vi "Add Subscriber.vi"(8 "error in (no error)":errorcluster, 10 "New FIFO Instance Config":T2 {"Custom Data" format="%.0x"}, 11 "CIF_CIPC_Chn in":refnum<class "CIF_Iceoryx_Chn.lvclass">) -> (0 "error out":errorcluster, 2 "New FIFO Instance":T1 {"Custom Data" format="%.0x"}, 3 "CIF_CIPC_Chn out":refnum<class "CIF_Iceoryx_Chn.lvclass">)   [LabVIEW 2021, in "CIF_Iceoryx_Chn.lvclass"]
uses:
  CIF_Iceoryx_Chn.lvclass
  CIF_Iceoryx_Chn.lvclass/CIF_Iceoryx_Chn.ctl
  ChannelCommon/typedef/New FIFO Instance Response.ctl
  ChannelCommon/ChannelCommon.lvlib
  CIFChannels/CIFChannels.lvclass
  D:/dev/Packages/CIF_Channels_Core/src/CIFChannels/CIFChannels.lvclass
  D:/dev/Packages/CIF_Channels_Core/src/Iceorxy_Channels/CIF_Iceoryx_Chan/CIF_Iceoryx_Chn.lvclass
  ChannelCommon/typedef/New FIFO Instance Configuration.ctl
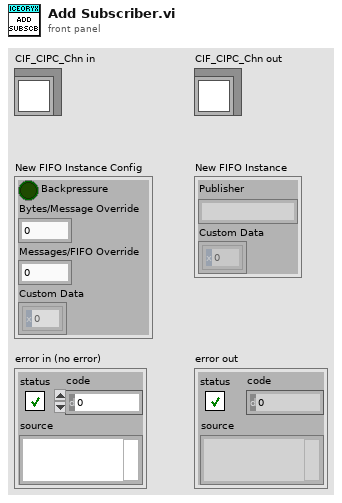
[diagram p1: front panel]
types:
  T1 = typedef "ChannelCommon.lvlib/New FIFO Instance Response.ctl" = cluster{"Publisher":string, "Custom Data":u8[]}
  T2 = typedef "ChannelCommon.lvlib/New FIFO Instance Configuration.ctl" = cluster{"Backpressure":bool, "Bytes/Message Override":u32, "Messages/FIFO Override":u32, "Custom Data":u8[]}
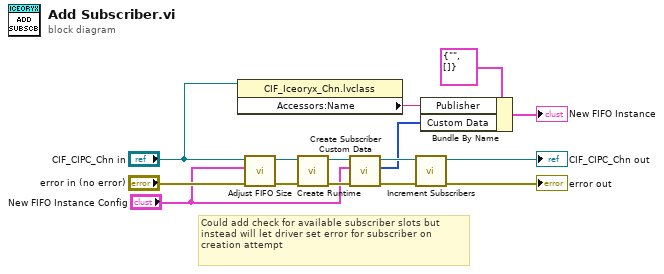
[diagram p0: block diagram]
diagram:
  # "Could add check for available subscriber slots but instead will let driver set error for subscriber on creation attempt"
  n1 = property class="CIF_Iceoryx_Chn.lvclass"(reference="CIF_CIPC_Chn in") -> ("Accessors:Name"=w7:string)  [unwired: 1 in, 2 out]
  n2 = call-dynamic "Adjust FIFO Size.vi"("error in (no error)"="error in (no error)", "New FIFO Instance Config"="New FIFO Instance Config", "CIF_CIPC_Chn in"="CIF_CIPC_Chn in") -> ("error out"=w8:errorcluster, "CIF_CIPC_Chn out"=w9:refnum<class "CIF_Iceoryx_Chn.lvclass">)  [unwired: 7 in]
  n3 = call-dynamic "Create Runtime.vi"("error in (no error)"=w8, "CIFChannels in"=w9) -> ("error out"=w5:errorcluster, "CIFChannels out"=w6:refnum<class "CIF_Iceoryx_Chn.lvclass">)  [unwired: 8 in]
  n4 = call-dynamic "Create Subscriber Custom Data.vi"("error in (no error)"=w5, "New FIFO Instance Config"="New FIFO Instance Config", "CIF_Iceoryx_Chan in"=w6) -> ("error out"=w4:errorcluster, "Custom Data"=w2:u8[], "CIF_Iceoryx_Chan out"=w3:refnum<class "CIF_Iceoryx_Chn.lvclass">)  [unwired: 6 in]
  n5 = call "Increment Subscribers.vi"("error in (no error)"=w4, "CIFChannels in"=w3) -> ("error out"=→"error out":errorcluster, "CIFChannels out"=→"CIF_CIPC_Chn out":refnum<class "CIF_Iceoryx_Chn.lvclass">)  [unwired: 8 in]
  n6 = Bundle By Name(cluster=T1 {"Publisher"="", "Custom Data"=[]} ("New FIFO Instance"), "Publisher"=w7, "Custom Data"=w2) -> (→"New FIFO Instance":T1)
